vi "XIS Get Latest Frame.vi"(7 "height":i32, 8 "error in (no error)":errorcluster, 9 "width":i32, 10 "bufferSize":i32, 11 "lvBuffer":u16) -> (0 "error out":errorcluster, 1 "width out":i32, 2 "function return":i32, 3 "lvBuffer out":u16, 5 "height out":i32)   [LabVIEW 2025, in "VarexWrapper.lvlib"]
doc: "VAREX_API int XIS_GetLatestFrame(\n unsigned short* lvBuffer,\n int bufferSize,\n int* width,\n int* height);"
uses:
  VarexWrapper.lvlib
  VarexWrapper.dll
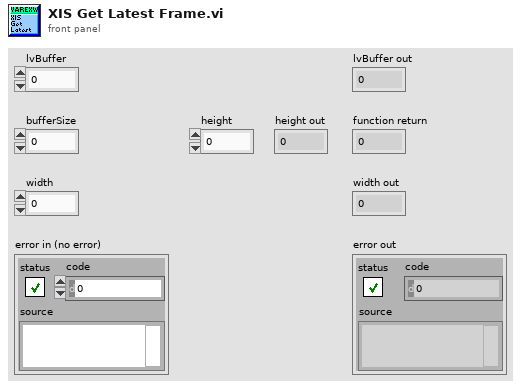
[diagram p1: front panel]
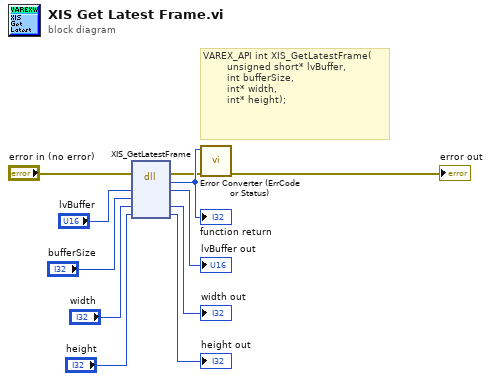
[diagram p0: block diagram]
diagram:
  # "VAREX_API int XIS_GetLatestFrame(\n        unsigned short* lvBuffer,\n        int bufferSize,\n        int* width,\n        int* height);"
  n1 = dll-call lib="C:/Users/AriNutpam User/Documents/GitHub/The-Oracle/Image Acquisition/Child Classes/VarexImager/VarexWrapperLvLib/VarexWrapper.*" fn="XIS_GetLatestFrame"(error in="error in (no error)", "lvBuffer"="lvBuffer", "bufferSize"="bufferSize", "width"="width", "height"="height") -> (error out=w2:errorcluster, w11:i32, "lvBuffer"=→"lvBuffer out":u16, "width"=→"width out":i32, "height"=→"height out":i32)  [unwired: 3 in, 1 out]
  "function return" <- w11
  n2 = call "Error Converter (ErrCode or Status).vi"("error in (no error)"=w2, "error code"=w11) -> ("error out"=→"error out":errorcluster)  [unwired: 9 in]
